vi "D_W_FMemBMPPath.vi"(8 "error in (no error)":errorcluster, 9 "slotNo":u32, 10 "BMP file path":path, 11 "bID":u8) -> (0 "error out":errorcluster, 3 "bID":u8, 4 "TorF":i32)   [LabVIEW 2013]
uses:
  LabVIEW2018/hpkSLMdaLV.dll
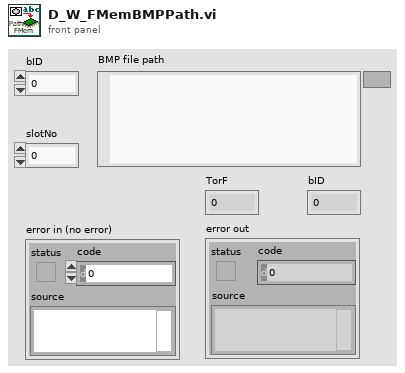
[diagram p1: front panel]
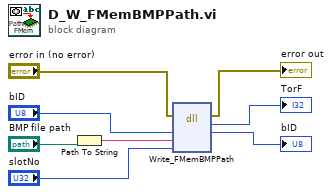
[diagram p0: block diagram]
diagram:
  n1 = Path To String(path="BMP file path") -> (string=w6:string)
  n2 = dll-call lib="C:/Users/hs5921/Desktop/LabVIEW2018/hpkSLMdaLV.dll" fn="Write_FMemBMPPath"(error in="error in (no error)", "bID"="bID", "path"=w6, "slotNo"="slotNo") -> (error out=→"error out":errorcluster, "返り値タイプ"=→"TorF":i32, "bID"=→"bID":u8)  [unwired: 4 in, 1 out]
